vi "VIH HelpGen - Image - Fill Region Around Point in 2D Array.vi"(8 "New Color (transparent)":u32(colorbox)=16777216, 10 "Point coords (0,0)":cluster{"row":i32, "col":i32}, 11 "Image Data in":u32[][](array[numeric]) format="%.0x") -> (0 "Replacements":i32, 3 "Image Data out":u32[][](array[numeric]) format="%.0x")   [LabVIEW 2014]
doc: "::: VI Helpeks :::\nCopyright (c) 2000-2026 Konstantin Shifershteyn. All rights reserved."
panel:
  out "max size":i32
  # "VI Helpeks\nCopyright (c) 2012-2026 Konstantin Shifershteyn"
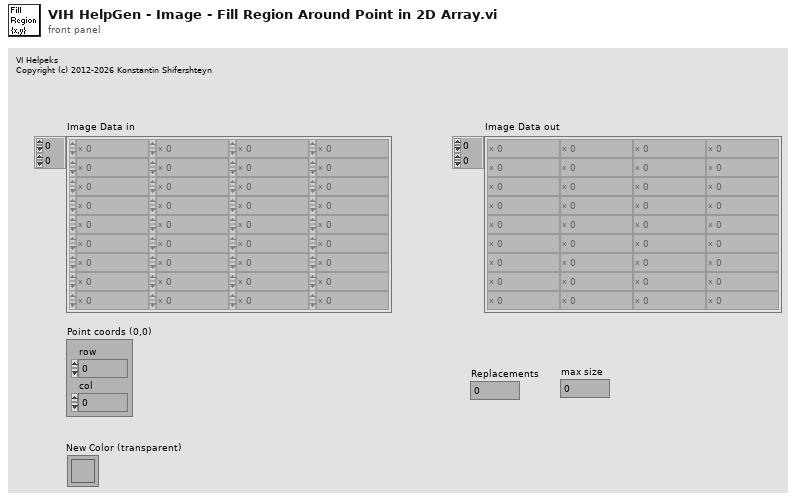
[diagram p1: front panel]
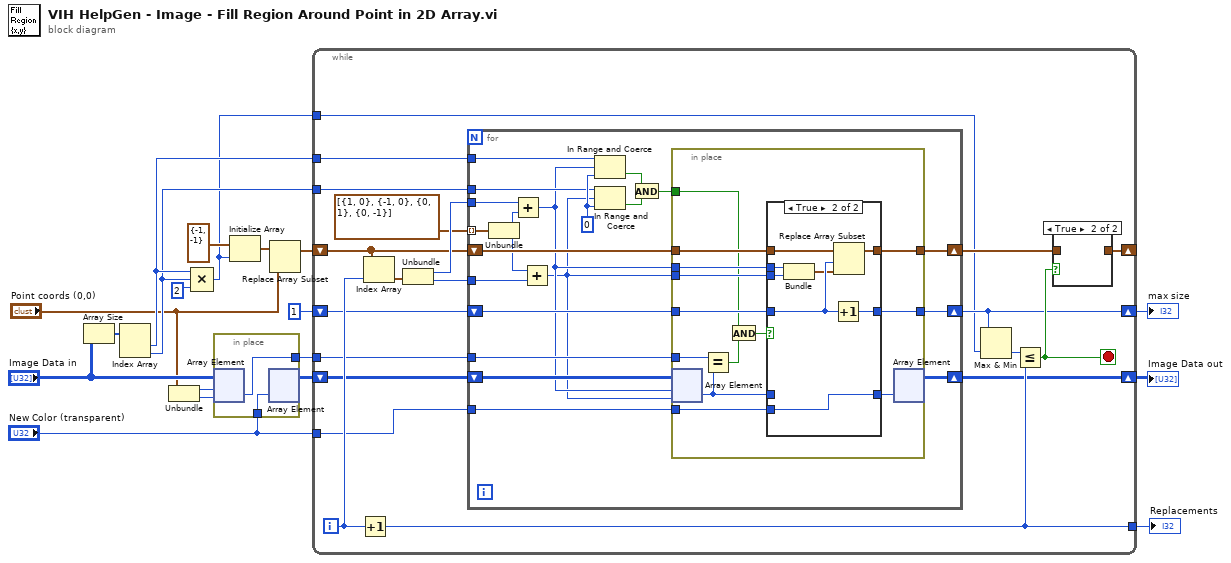
[diagram p0: block diagram]
diagram:
  n1 = Array Size(array="Image Data in") -> (size(s)=w18:i32[])
  n2 = Index Array(array=w18) -> (element #1=w16:i32, element #2=w11:i32)  [unwired: 2 in]
  n3 = Unbundle("Point coords (0,0)") -> ("row"=w7:i32, "col"=w6:i32)
  n4 = Compound Arithmetic op=MULTIPLY(w16, w11, 2 ("y")) -> (w1:i32)
  n5 = in-place {
    in-place-border: [w21] -> w4
    in-place-border: "New Color (transparent)" -> [w20]
    n6 = in-place-array #1("Image Data in", w7, w6) -> (w21:u32)
    n7 = in-place-array #1(w20) -> (w8:u32[][])  [unwired: 2 out]
  }
  n8 = Initialize Array(cluster{i32, i32} {-1, -1} ("output cluster"), w1) -> (w15:cluster{i32, i32}[])
  n9 = Replace Array Subset(array=w15, new element="Point coords (0,0)") -> (w14:cluster{i32, i32}[])  [unwired: 1 in]
  n10 = while {
    shift-right: [w26] -> w19
    shift-left: w8 -> [w25]
    shift-right: [w35] -> _
    shift-left: w14 -> [w40]
    tunnel: [w36] -> w2
    tunnel: w16 -> [w32]
    tunnel: w11 -> [w31]
    shift-right: [w23] -> w12
    shift-left: 1 -> [w30]
    tunnel: "New Color (transparent)" -> [w27]
    tunnel: w4 -> [w29]
    tunnel: w1 -> [w22]
    i -> [w39]
    stop <- w34 stop-if-true
    n11 = Increment(x=w39) -> (x+1=w36:i32)
    n12 = Index Array(array=w40, index=w39) -> (element=w38:cluster{i32, i32})
    n13 = Unbundle(w38) -> (w41:i32, w28:i32)
    n14 = for {
      tunnel: cluster{i32, i32}[] [{1, 0}, {-1, 0}, {0, 1}, {0, -1}] -> [w62] mode=indexing
      tunnel: w41 -> [w60]
      tunnel: w32 -> [w58]
      tunnel: w31 -> [w57]
      shift-right: [w55] -> w37
      shift-left: w40 -> [w56]
      shift-right: [w52] -> w23
      shift-left: w30 -> [w51]
      tunnel: w29 -> [w46]
      tunnel: w28 -> [w49]
      shift-right: [w47] -> w26
      shift-left: w25 -> [w48]
      tunnel: w27 -> [w45]
      w59 = 0 ("lower limit")
      n15 = Unbundle(w62) -> (w61:i32, w50:i32)
      n16 = Add(x=w60, y=w61) -> (x+y=w44:i32)
      n17 = Add(x=w50, y=w49) -> (x+y=w43:i32)
      n18 = In Range and Coerce(upper limit=w58, x=w44, lower limit=w59) -> (In Range?=w54:bool)  [unwired: 1 out]
      n19 = In Range and Coerce(upper limit=w57, x=w43, lower limit=w59) -> (In Range?=w53:bool)  [unwired: 1 out]
      n20 = And(x=w54, y=w53) -> (x .and. y?=w42:bool)
      n21 = in-place {
        in-place-border: w56 -> [w75]
        in-place-border: [w74] -> w55
        in-place-border: [w73] -> w52
        in-place-border: w51 -> [w72]
        in-place-border: w46 -> [w71]
        in-place-border: w45 -> [w68]
        in-place-border: w44 -> [w67]
        in-place-border: w43 -> [w66]
        in-place-border: w42 -> [w64]
        n22 = in-place-array #2(w48, w44, w43) -> (w69:u32)
        n23 = Equal?(x=w71, y=w69) -> (x = y?=w65:bool)
        n24 = And(x=w64, y=w65) -> (x .and. y?=w63:bool)
        n25 = case shown="True" w63 {
          tunnel: w75 -> [w78 w86]
          tunnel: [w78 w85] -> w74
          tunnel: [w77 w84] -> w73
          tunnel: w72 -> [w77 w83]
          tunnel: w67 -> [_ w82]
          tunnel: w66 -> [_ w81]
          tunnel: [w76 w79] -> w70
          tunnel: w69 -> [w76 _]
          tunnel: w68 -> [_ w79]
          frame False {
          }
          frame True {
            n26 = Bundle(w82, w81) -> (w80:cluster{i32, i32})  [unwired: 1 in]
            n27 = Increment(x=w83) -> (x+1=w84:i32)
            n28 = Replace Array Subset(array=w86, new element=w80, index=w83) -> (w85:cluster{i32, i32}[])
          }
        }
        n29 = in-place-array #2(w70) -> (w47:u32[][])  [unwired: 2 out]
      }
    }
    n30 = Max & Min(x=w23, y=w22) -> (min(x,y)=w24:i32)  [unwired: 1 out]
    n31 = Less Or Equal?(x=w24, y=w36) -> (x <= y?=w34:bool)
    n32 = case shown="True" w34 {
      tunnel: w37 -> [w87 _]
      tunnel: [w87 _] -> w35
      frame False {
      }
      frame True {
      }
    }
  }
  "Image Data out" <- w19
  "Replacements" <- w2
  "max size" <- w12
